vi "IMU Get Yaw Landscapevi.vi"(7 "Set Yaw Angle":dbl=nan, 8 "error in (no error)":errorcluster, 10 "Units":enum16{"Radians", "Degrees"}(ring)) -> (0 "error out":errorcluster, 2 "timestamp out":i64, 3 "yaw":dbl(graph))   [LabVIEW 2023, in "MrcLib.lvlib"]
doc: "Return the yaw of the built-in sensor in the indicated units assuming it is mounted vertically with long edge parallel to the ground (somewhat common). To align with a existing coordinate system, make a call passing in the expected alignment angle."
uses:
  <vilib>/MRC/MrcLib.lvlib
  <vilib>/MRC/MrcLib/VIs/IMU/MRC IMU Get Yaw Landscape.vi
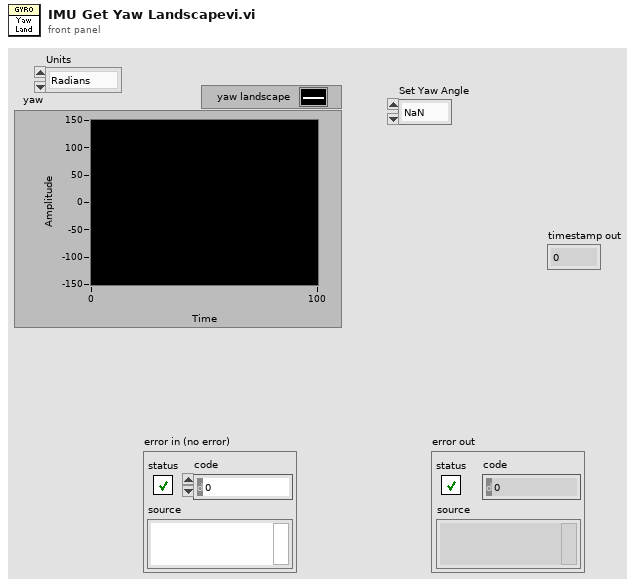
[diagram p1: front panel]
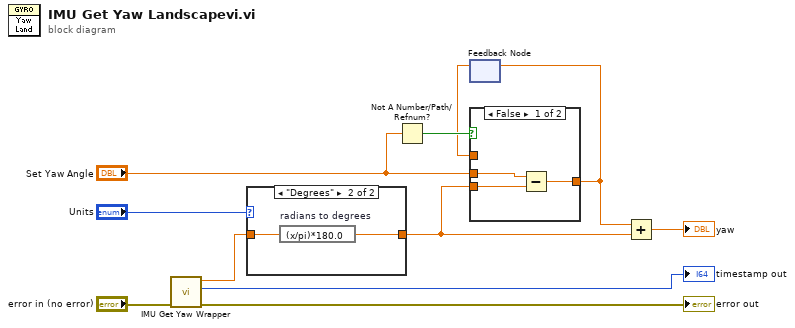
[diagram p0: block diagram]
diagram:
  n1 = call-poly <vilib>:"IMU Get Yaw Wrapper.vi"("error in (no error)"="error in (no error)") -> ("error out"=→"error out":errorcluster, "timestamp out"=→"timestamp out":i64, "yaw out"=w2:dbl)  [unwired: 7 in, 1 out]
  n2 = case shown="\"Degrees\"" "Units" {
    tunnel: w2 -> [w12 w14]
    tunnel: [w12 w13] -> w3
    frame "Radians", Default {
    }
    frame "Degrees" {
      n3 = expression code="(x/pi)*180.0" "radians to degrees"(w14) -> (w13:dbl)
    }
  }
  n4 = Not A Number/Path/Refnum?(number/path/refnum="Set Yaw Angle") -> (NaN/Path/Refnum?=w8:bool)
  n5 = feedback #1() -> (w7:dbl)  [unwired: 1 in]
  n6 = case shown="False" w8 {
    tunnel: w3 -> [w17 _]
    tunnel: "Set Yaw Angle" -> [w16 _]
    tunnel: [w15 w18] -> w6
    tunnel: w7 -> [_ w18]
    frame False {
      n7 = Subtract(x=w16, y=w17) -> (x-y=w15:dbl)
    }
    frame True {
    }
  }
  n8 = feedback-in #1(w6) -> ()
  n9 = Add(x=w6, y=w3) -> (x+y=→"yaw":dbl)
